vi "Look for Control And Get Parameter.vi"(10 "Label":string, 11 "VIs.Ctrls":T1[](array[typedef])) -> (0 "Used CTRL":bool, 1 "Use in VIs":string[](array[string]), 2 "Class Name":string, 3 "Selected CTRLs":T1[](array[typedef]), 4 "Caption Is Vissible":bool)   [LabVIEW 2019, in "Language Editor.lvlib"]
doc: "- - -\nCopyright (c) 2026, Merecs Engineering GmbH"
uses:
  Language Editor.lvlib
  type defs/Cluster VI controls.ctl
panel:
  # "Connector Pane"
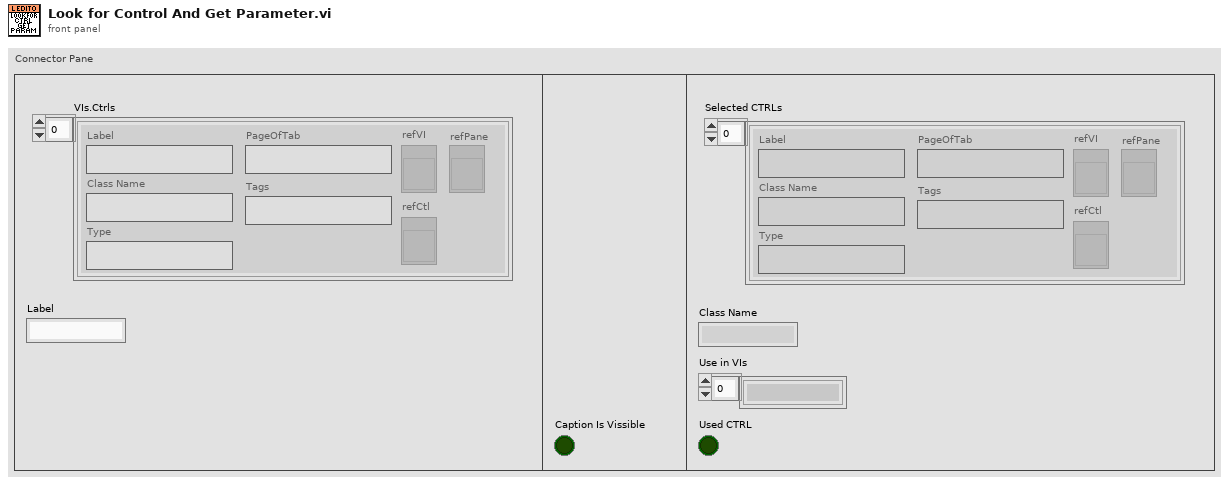
[diagram p1: front panel]
types:
  T1 = typedef "Language Editor.lvlib/Cluster VI controls.ctl" = cluster{"Label":string, "Class Name":string, "Type":string, "Tags":string, "refVI":refnum<vi>, "refCtl":refnum<vi>, "PageOfTab":string, "refPane":refnum<vi>}
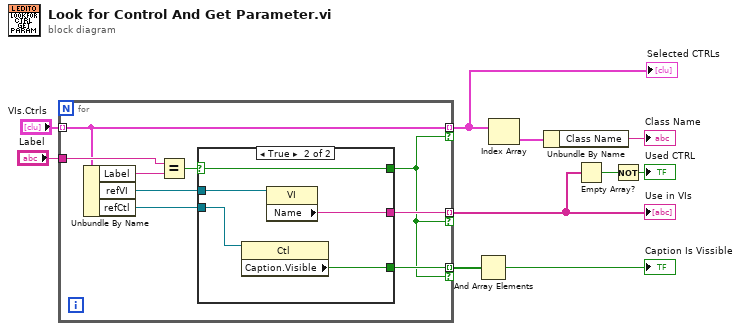
[diagram p0: block diagram]
diagram:
  n1 = for {
    tunnel: "VIs.Ctrls" -> [w17] mode=indexing
    tunnel: "Label" -> [w18]
    tunnel: [w17] -> w6 mode=indexing if=w11
    tunnel: [w13] -> w3 mode=indexing if=w11
    tunnel: [w12] -> w5 mode=indexing if=w11
    n2 = Unbundle By Name(w17) -> ("Label"=w19:string, "refVI"=w15:refnum<vi>, "refCtl"=w14:refnum<vi>)
    n3 = Equal?(x=w18, y=w19) -> (x = y?=w16:bool)
    n4 = case shown="True" w16 {
      selector: w16 -> [_ w24]
      tunnel: [_ w24] -> w11
      tunnel: w15 -> [_ w22]
      tunnel: w14 -> [_ w23]
      tunnel: [_ w21] -> w13
      tunnel: [_ w20] -> w12
      frame False {
      }
      frame True {
        n5 = property class="Ctl"(reference=w23) -> ("Caption.Visible"=w20:bool)  [unwired: 1 in, 2 out]
        n6 = property class="VI"(reference=w22) -> ("Name"=w21:string)  [unwired: 1 in, 2 out]
      }
    }
  }
  "Use in VIs" <- w3
  "Selected CTRLs" <- w6
  n7 = And Array Elements(Boolean array=w5) -> (logical AND=→"Caption Is Vissible":bool)
  n8 = Index Array(array=w6) -> (element=w10:T1)  [unwired: 1 in]
  n9 = Unbundle By Name(w10) -> ("Class Name"=→"Class Name":string)
  n10 = Empty Array?(array=w3) -> (empty?=w2:bool)
  n11 = Not(x=w2) -> (.not. x?=→"Used CTRL":bool)
